vi "query OBW Measurement Result.vi"(8 "error in (no error)":errorcluster, 11 "FSV-40N in":refnum<class "FSV-40N.lvclass">) -> (0 "error out":errorcluster, 2 "OBW Measurement":T1, 3 "FSV-40N out":refnum<class "FSV-40N.lvclass">)   [LabVIEW 2023, in "Spectrum Analyzer.lvlib" / "FSV-40N.lvclass"]
uses:
  FSV-40N.lvclass
  TYPE DEFINITION/SA Measurement Class/TYPE OBW Measurement.ctl
  Spectrum Analyzer.lvlib
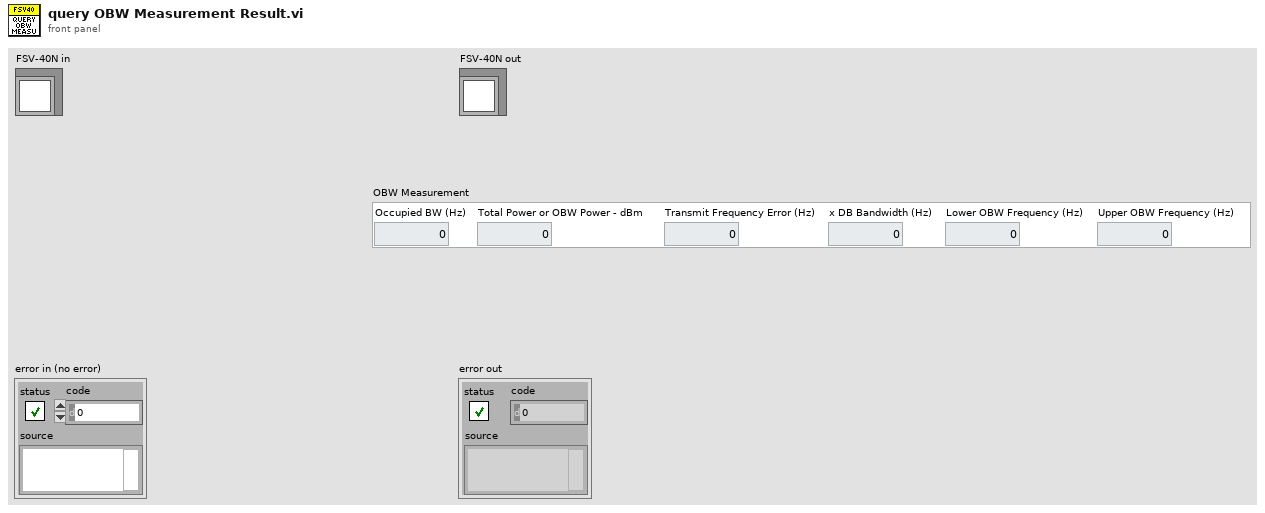
[diagram p1: front panel]
types:
  T1 = typedef "Spectrum Analyzer.lvlib/TYPE OBW Measurement.ctl" = cluster{"Occupied BW (Hz)":dbl, "Total Power or OBW Power - dBm":dbl, "Transmit Frequency Error (Hz)":dbl, "x DB Bandwidth (Hz)":dbl, "Lower OBW Frequency (Hz)":dbl, "Upper OBW Frequency (Hz)":dbl}
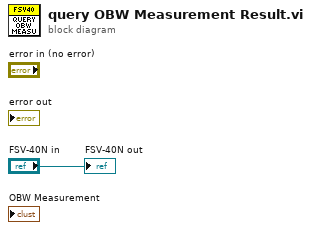
[diagram p0: block diagram]
diagram:
  "FSV-40N out" <- "FSV-40N in"
